vi "G4BaseTemplate_Singleton_6x8x6_WriteAttribute.vi"(5 "Error In":errorcluster) -> (19 "Error Out":errorcluster)   [LabVIEW 2020]
uses:
  G4BaseTemplate_Singleton_6x8x6.lvclass
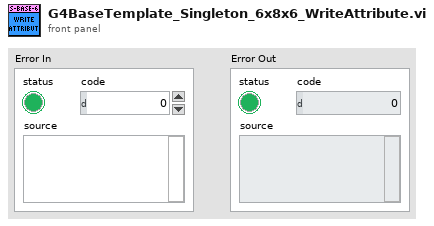
[diagram p1: front panel]
types:
  T1 = typedef "G4BaseTemplate_Singleton_6x8x6.lvclass/ObjectAttributes.ctl" = cluster{"Attribute1":dbl}
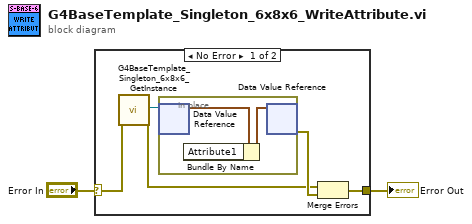
[diagram p0: block diagram]
diagram:
  n1 = case shown="No Error" "Error In" {
    selector: "Error In" -> [w7 w10]
    tunnel: [w3 w10] -> w1
    frame No Error {
      n2 = call "G4BaseTemplate_Singleton_6x8x6_GetInstance.vi"("Error In"=w7) -> ("DVRRefOut"=w5:refnum<data-value>, "Error Out"=w4:errorcluster)  [unwired: 14 in, 3 out]
      n3 = in-place {
        n4 = in-place-dvr #1(w5) -> (w8:T1)  [unwired: 1 out]
        n5 = Bundle By Name(cluster=w8) -> (w9:T1)  [unwired: 1 in]
        n6 = in-place-dvr #1(w9) -> (w6:errorcluster)  [unwired: 1 out]
      }
      n7 = Merge Errors(w4, w6) -> (w3:errorcluster)
    }
    frame Error {
    }
  }
  "Error Out" <- w1
